vi "Waveform Inputs.vi"(8 "error in (no error)":errorcluster, 11 "Node Ptr":T1 format="%.0x") -> (0 "error out":errorcluster)   [LabVIEW 2020, in "FPGA Addon System Explorer.lvlib"]
uses:
  FPGA Addon System Explorer.lvlib
  <vilib>/NI VeriStand/Custom Device API/Custom Device API.lvlib
  Types/Channel Type.ctl
  Types/SE UI Cluster.ctl
  <vilib>/NI VeriStand/Custom Device API/Custom Device Item Ref.ctl
panel:
  in  "remove":bool
  in  "add":bool
  in  "Available Registers":i32[](listbox)
  in  "Header 2":cluster{"Section Name":string}={"Section Name"="Register Settings"}
  in  "SHDocVw.IWebBrowser":refnum<k7>(container)
  in  "Header":cluster{"Section Name":string}={"Section Name"="Section Settings"}
  in  "Description":string
  out "Name":string
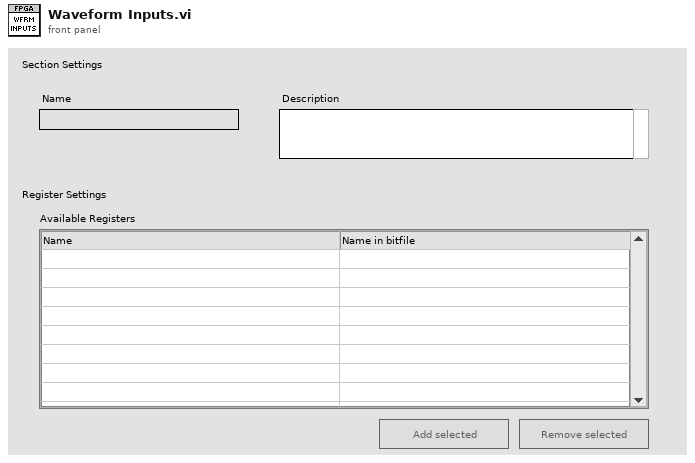
[diagram p1: front panel]
types:
  T1 = typedef "Custom Device API.lvlib/Custom Device Item Ref.ctl" = u64
  T2 = typedef "FPGA Addon System Explorer.lvlib/SE UI Cluster.ctl" = cluster{"Node Ptr":T1, "Add":refnum<vi>, "Remove":refnum<vi>, "Registers ListBox":refnum<vi>}
  T3 = typedef "Custom Device API.lvlib/Custom Device Item Info.ctl" = cluster{"Name":string, "Is Channel":bool, "GUID":string, "Is Waveform":bool}
  T4 = typedef "FPGA Addon System Explorer.lvlib/Channel Type.ctl" = enum16{"Write Channel", "Read Channel", "Write Waveform", "Read Waveform"}
  T5 = typedef "Custom Device API.lvlib/Custom Device Commands.ctl" = enum16{"Default", "Item renamed", "Shutdown", "Dynamic button pressed"}
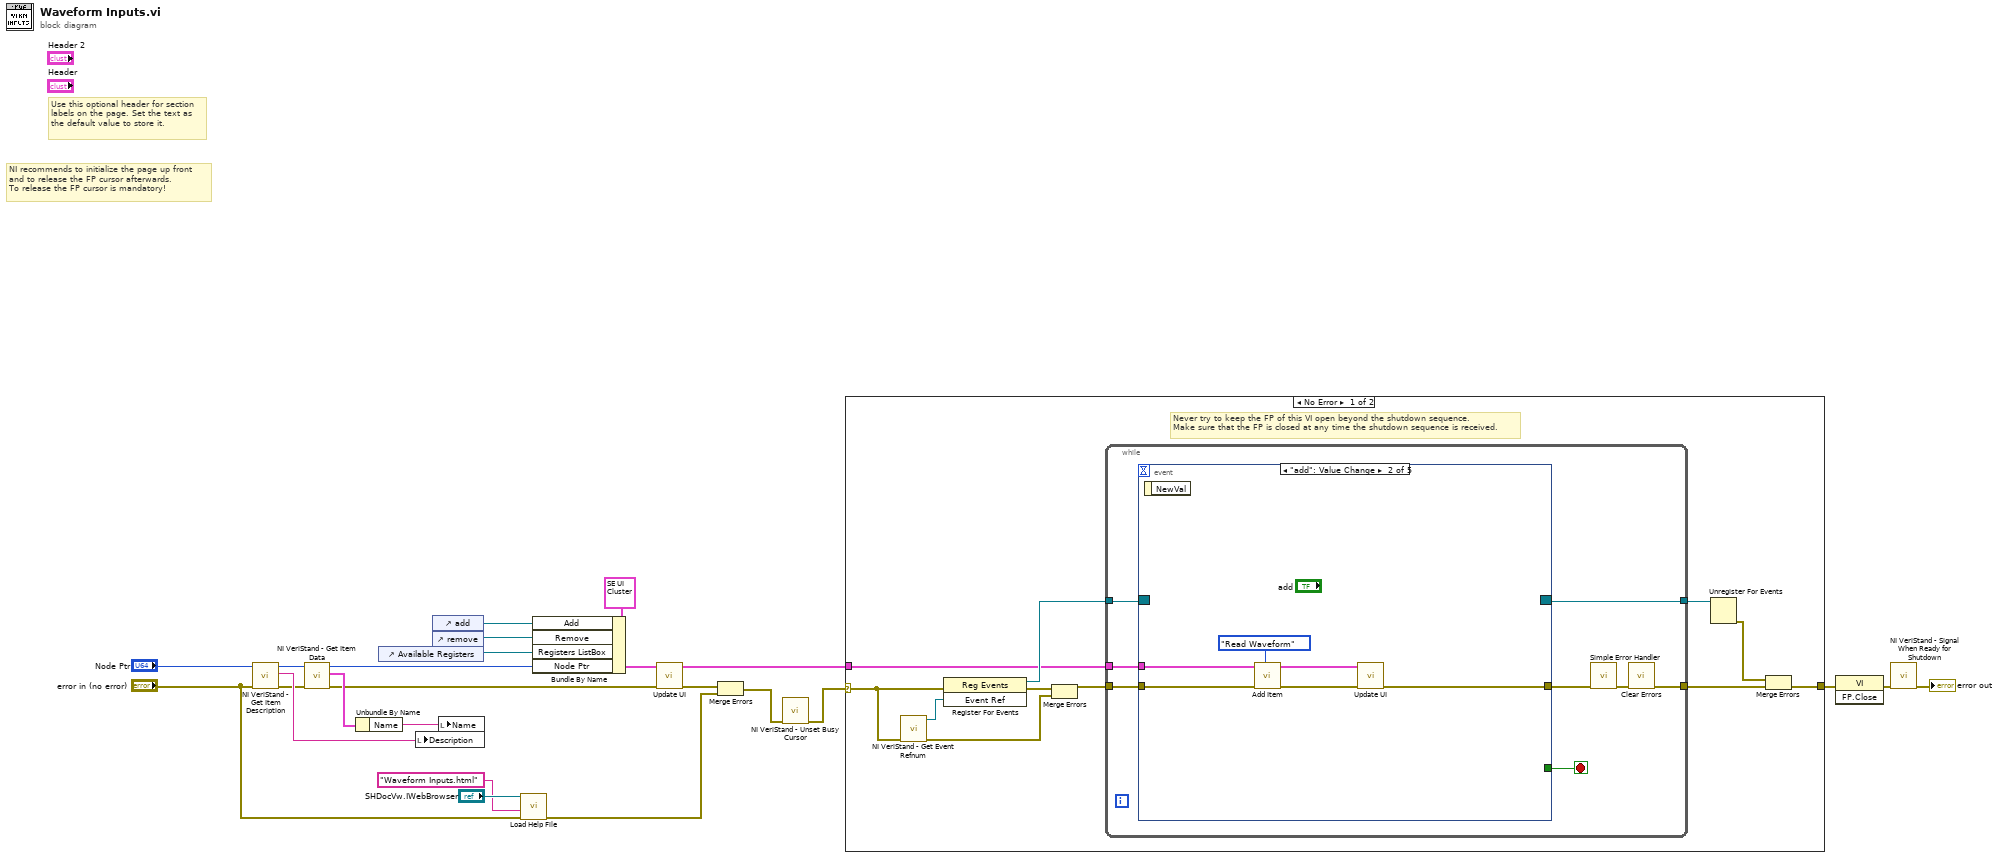
[diagram p0: block diagram]
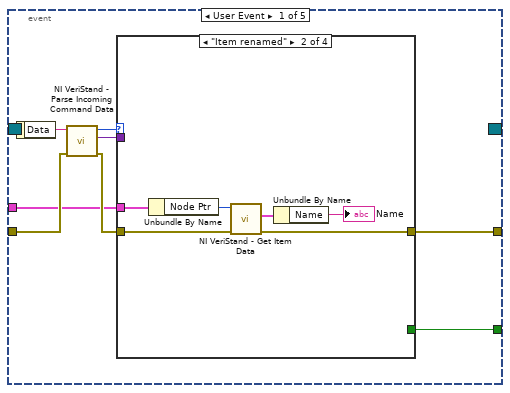
[diagram p2: hidden frame]
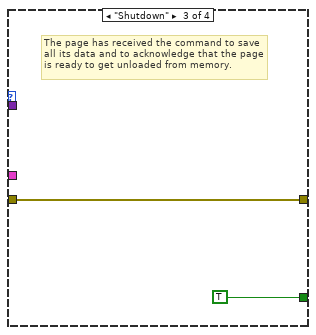
[diagram p4: hidden frame]
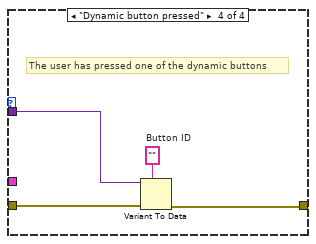
[diagram p5: hidden frame]
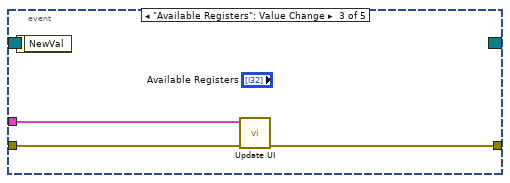
[diagram p6: hidden frame]
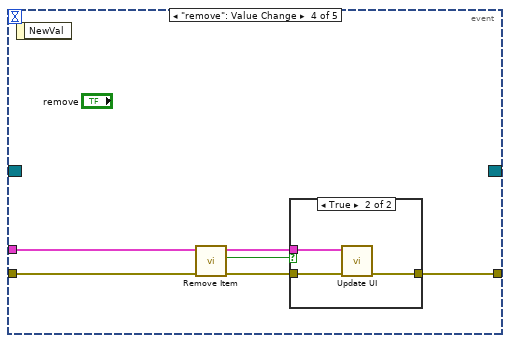
[diagram p7: hidden frame]
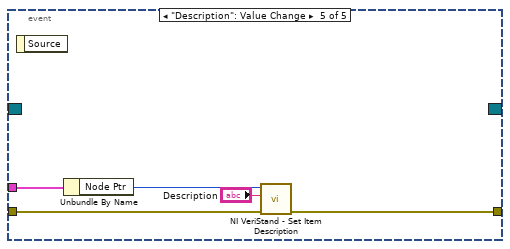
[diagram p9: hidden frame]
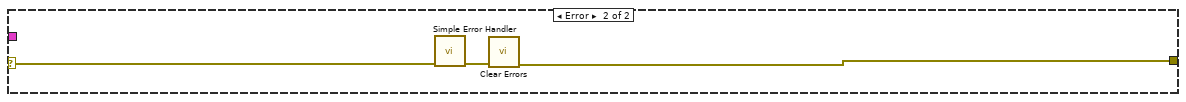
[diagram p10: hidden frame]
diagram:
  # "Use this optional header for section labels on the page. Set the text as the default value to store it."
  # "NI recommends to initialize the page up front\nand to release the FP cursor afterwards.\nTo release the FP cursor is mandatory!"
  n1 = call <vilib>:"NI VeriStand - Get Item Description.vi"("error in (no error)"="error in (no error)", "Item Ref in"="Node Ptr") -> ("error out"=w15:errorcluster, "Description"=w16:string, "Item Ref out"=w17:T1)  [unwired: 7 out]
  n2 = call <vilib>:"NI VeriStand - Get Item Data.vi"("error in (no error)"=w15, "Item Ref in"=w17) -> ("error out"=w12:errorcluster, "Item Info"=w14:T3, "Item Ref out"=w7:T1)  [unwired: 7 out]
  n3 = Unbundle By Name(w14) -> ("Name"=w13:string)
  n4 = control-ref of="Available Registers"() -> (w11:refnum<vi>)
  n5 = local write "Description"(w16) -> ()
  n6 = control-ref of="add"() -> (w10:refnum<vi>)
  n7 = control-ref of="remove"() -> (w9:refnum<vi>)
  n8 = local write "Name"(w13) -> ()
  n9 = call "Load Help File.vi"("error in (no error)"="error in (no error)", "HTML File to Load"="Waveform Inputs.html" ("HTML File"), "SHDocVw.IWebBrowser2"="SHDocVw.IWebBrowser") -> ("error out"=w4:errorcluster)  [unwired: 8 in]
  n10 = Bundle By Name(cluster=T2 {"Node Ptr"=18446744073709551615, "Add"=refnum, "Remove"=refnum, "Registers ListBox"=refnum} ("SE UI Cluster"), "Add"=w10, "Remove"=w9, "Registers ListBox"=w11, "Node Ptr"=w7) -> (w6:T2)
  n11 = call "Update UI.vi"("error in (no error)"=w12, "SE UI cluster in"=w6) -> ("error out"=w5:errorcluster, "SE UI cluster out"=w3:T2)  [unwired: 8 in]
  n12 = Merge Errors(w5, w4) -> (w2:errorcluster)
  n13 = call <vilib>:"NI VeriStand - Unset Busy Cursor.vi"("error in (no error)"=w2) -> ("error out"=w1:errorcluster)  [unwired: 10 out]
  n14 = case shown="No Error" w1 {
    selector: w1 -> [w32 w91]
    tunnel: [w25 w89] -> w24
    tunnel: w3 -> [w29 _]
    frame No Error {
      # "Never try to keep the FP of this VI open beyond the shutdown sequence.\nMake sure that the FP is closed at any time the shutdown sequence is received."
      n15 = call <vilib>:"NI VeriStand - Get Event Refnum.vi"("error in (no error)"=w32) -> ("error out"=w31:errorcluster, "Event Ref"=w33:refnum<user-event>)  [unwired: 9 out]
      n16 = register-events(error in=w32, w33) -> (reference out=w34:refnum<event-registration>, error out=w30:errorcluster)  [unwired: 1 in]
      n17 = Merge Errors(w30, w31) -> (w28:errorcluster)
      n18 = while {
        tunnel: w29 -> [w40]
        tunnel: w28 -> [w39]
        tunnel: w34 -> [w42]
        tunnel: [w43] -> w35
        tunnel: [w36] -> w27
        stop <- w41 stop-if-true
        n19 = event shown="[1] \"add\": Value Change" {
          selector: w42 -> [_ _ _ _ _]
          dyn-events: [_ _ _ _ _] -> w43
          timeout: _ -> [_ _ _ _ _]
          tunnel: [w48 _ _ _ _] -> w41
          tunnel: [w47 w66 w71 w76 w88] -> w37
          tunnel: w40 -> [w44 w69 w72 w78 w86]
          tunnel: w39 -> [w45 w68 w73 w79 w85]
          event User Event {
            n20 = event-data() -> ("Data"=w51:string)  [unwired: 1 out]
            n21 = call <vilib>:"NI VeriStand - Parse Incoming Command Data.vi"("error in (no error)"=w45, "Incoming data"=w51) -> ("error out"=w50:errorcluster, "Outgoing data"=w46:variant, "Action"=w49:T5)  [unwired: 7 out]
            n22 = case shown="\"Item renamed\"" w49 {
              tunnel: w50 -> [w52 w58 w59 w64]
              tunnel: [_ _ TRUE _] -> w48
              tunnel: [w52 w56 w59 w61] -> w47
              tunnel: w46 -> [_ _ _ w63]
              tunnel: w44 -> [_ w53 _ _]
              frame "Default", Default {
              }
              frame "Item renamed" {
                n23 = Unbundle By Name(w53) -> ("Node Ptr"=w55:T1)
                n24 = call <vilib>:"NI VeriStand - Get Item Data.vi"("error in (no error)"=w58, "Item Ref in"=w55) -> ("error out"=w56:errorcluster, "Item Info"=w57:T3)  [unwired: 8 out]
                n25 = Unbundle By Name(w57) -> ("Name"=→"Name":string)
              }
              frame "Shutdown" {
                # "The page has received the command to save all its data and to acknowledge that the page is ready to get unloaded from memory."
              }
              frame "Dynamic button pressed" {
                w62 = ""  # Button ID
                # "The user has pressed one of the dynamic buttons"
                n26 = Variant To Data(error in=w64, type=w62, Variant=w63) -> (error out=w61:errorcluster)  [unwired: 1 out]
              }
            }
          }
          event "add": Value Change {
            n27 = event-data() -> ()  [unwired: 2 out]
            n28 = call "Add Item.vi"("Action"=Channel_Type."Read Waveform", "error in (no error)"=w68, "SE UI cluster in"=w69) -> ("error out"=w67:errorcluster, "SE UI cluster out"=w65:T2)  [unwired: 7 in]
            n29 = call "Update UI.vi"("error in (no error)"=w67, "SE UI cluster in"=w65) -> ("error out"=w66:errorcluster)  [unwired: 8 in, 1 out]
          }
          event "Available Registers": Value Change {
            n30 = event-data() -> ()  [unwired: 2 out]
            n31 = call "Update UI.vi"("error in (no error)"=w73, "SE UI cluster in"=w72) -> ("error out"=w71:errorcluster)  [unwired: 8 in, 1 out]
          }
          event "remove": Value Change {
            n32 = event-data() -> ()  [unwired: 2 out]
            n33 = call "Remove Item.vi"("error in (no error)"=w79, "SE UI cluster in"=w78) -> ("error out"=w77:errorcluster, "Deleted?"=w74:bool, "SE UI cluster out"=w75:T2)  [unwired: 7 in]
            n34 = case shown="True" w74 {
              tunnel: w77 -> [w80 w83]
              tunnel: [w80 w82] -> w76
              tunnel: w75 -> [_ w81]
              frame False {
              }
              frame True {
                n35 = call "Update UI.vi"("error in (no error)"=w83, "SE UI cluster in"=w81) -> ("error out"=w82:errorcluster)  [unwired: 8 in, 1 out]
              }
            }
          }
          event "Description": Value Change {
            n36 = event-data() -> ()  [unwired: 2 out]
            n37 = Unbundle By Name(w86) -> ("Node Ptr"=w84:T1)
            n38 = call <vilib>:"NI VeriStand - Set Item Description.vi"("error in (no error)"=w85, "Description"="Description", "Item Ref in"=w84) -> ("error out"=w88:errorcluster)  [unwired: 8 out]
          }
        }
        n39 = call <vilib>:"Simple Error Handler.vi"("error in (no error)"=w37) -> ("error out"=w38:errorcluster)  [unwired: 1 in, 7 out]
        n40 = call <vilib>:"Clear Errors.vi"("error in (no error)"=w38) -> ("error out"=w36:errorcluster)  [unwired: 1 in, 5 out]
      }
      n41 = Unregister For Events(event registration refnum=w35) -> (error out=w26:errorcluster)  [unwired: 1 in]
      n42 = Merge Errors(w26, w27) -> (w25:errorcluster)
    }
    frame Error {
      n43 = call <vilib>:"Simple Error Handler.vi"("error in (no error)"=w91) -> ("error out"=w90:errorcluster)  [unwired: 1 in, 7 out]
      n44 = call <vilib>:"Clear Errors.vi"("error in (no error)"=w90) -> ("error out"=w89:errorcluster)  [unwired: 1 in, 5 out]
    }
  }
  n45 = invoke class="VI" method="FP.Close"(error in=w24) -> (error out=w23:errorcluster)  [unwired: 2 in, 2 out]
  n46 = call <vilib>:"NI VeriStand - Signal When Ready for Shutdown.vi"("error in (no error)"=w23) -> ("error out"=→"error out":errorcluster)  [unwired: 10 out]
